vi "Replace String in File.vi"(7 "File Path":path, 8 "error in":errorcluster, 9 "Replace String":string, 10 "Search String":string, 11 "File Manager in":refnum<class "File Manager.lvclass">) -> (0 "error out":errorcluster, 3 "File Manager out":refnum<class "File Manager.lvclass">)   [LabVIEW 2026, in "File Manager.lvclass"]
doc: "This VI replaces all instances of the search string by the replace strin in the provided text file."
uses:
  File Manager.lvclass
  File Manager.lvclass/File Manager.ctl
  Interfaces/ILogger/ILogger Messages/Log Msg/Log Msg.lvclass/Log Msg.ctl
  <vilib>/ActorFramework/Message Enqueuer/Message Enqueuer.lvclass/Message Enqueuer.ctl
  <vilib>/ActorFramework/Message Enqueuer/Enqueue.vi
  Interfaces/ILogger/ILogger Messages/Log Msg/Log Msg.lvclass
  <vilib>/ActorFramework/Message Priority Queue/Priority Enqueue.vi
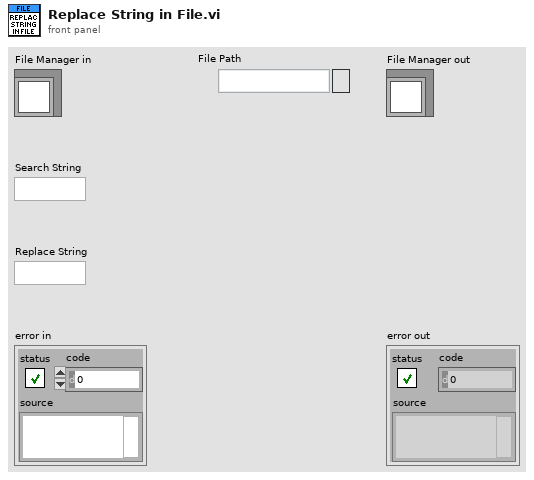
[diagram p1: front panel]
types:
  T1 = enum16{"open", "replace", "create", "open or create", "replace or create", "replace or create with confirmation"}
  T2 = typedef "Log Entry--cluster.ctl" = cluster{"Time":timestamp, "Message":string}
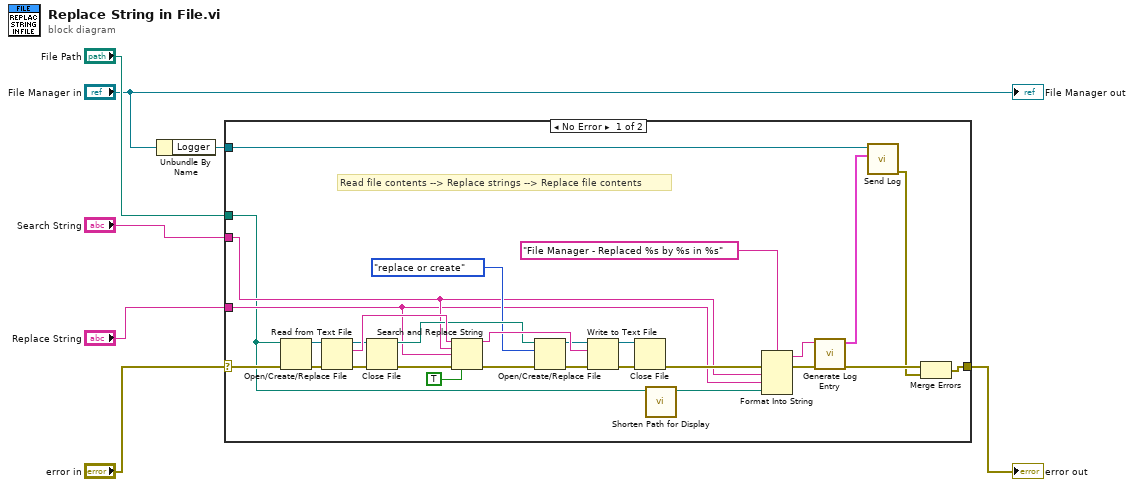
[diagram p0: block diagram]
diagram:
  n1 = Unbundle By Name("File Manager in") -> ("Logger"=w1:refnum<class "Message Enqueuer.lvclass">)
  n2 = case shown="No Error" "error in" {
    selector: "error in" -> [w30 w37]
    tunnel: "File Path" -> [w8 _]
    tunnel: "Search String" -> [w12 _]
    tunnel: "Replace String" -> [w11 _]
    tunnel: [w26 w37] -> w7
    tunnel: w1 -> [w15 _]
    frame No Error {
      # "Read file contents --> Replace strings --> Replace file contents"
      n3 = Open/Create/Replace File(file path (use dialog)=w8, error in=w30) -> (refnum out=w24:refnum<file>, error out=w36:errorcluster)  [unwired: 4 in, 1 out]
      n4 = Read from Text File(file (use dialog)=w24, error in=w36) -> (refnum out=w19:refnum<file>, text=w23:string, error out=w34:errorcluster)  [unwired: 2 in, 1 out]
      n5 = Close File(refnum=w19, error in=w34) -> (path=w18:path, error out=w33:errorcluster)
      n6 = Search and Replace String(replace all?=TRUE ("replace all? (F)"), input string=w23, search string=w12, replace string=w11, error in=w33) -> (result string=w21:string, error out=w32:errorcluster)  [unwired: 3 in, 2 out]
      n7 = Open/Create/Replace File(file path (use dialog)=w18, error in=w32, operation (0:open)=T1."replace or create") -> (refnum out=w17:refnum<file>, error out=w31:errorcluster)  [unwired: 3 in, 1 out]
      n8 = Write to Text File(file (use dialog)=w17, text=w21, error in=w31) -> (refnum out=w20:refnum<file>, error out=w35:errorcluster)  [unwired: 1 in, 1 out]
      n9 = Close File(refnum=w20, error in=w35) -> (error out=w28:errorcluster)  [unwired: 1 out]
      n10 = call "Shorten Path for Display.vi"("Path"=w8) -> ("Shortened Path"=w9:path)  [unwired: 10 in]
      n11 = Format Into String(format string="File Manager - Replaced %s by %s in %s", error in=w28, w12, w11, w9) -> (resulting string=w13:string, error out=w27:errorcluster)  [unwired: 1 in]
      n12 = call "Generate Log Entry.vi"("error in"=w27, "Message"=w13) -> ("error out"=w29:errorcluster, "Log Entry"=w10:T2)  [unwired: 8 in]
      n13 = call "Send Log.vi"("Log Entry"=w10, "Message Enqueuer"=w15) -> ("error out"=w25:errorcluster)  [unwired: 8 in, 1 out]
      n14 = Merge Errors(w29, w25) -> (w26:errorcluster)
    }
    frame Error {
      # "Pass error without further action."
    }
  }
  "error out" <- w7
  "File Manager out" <- "File Manager in"
